vi "LOGIN_rev-1 - Copy.vi"(8 "error in (no error)":errorcluster) -> (0 "error out":errorcluster)   [LabVIEW 2021]
uses:
  Control/login_type.ctl
  Control/User_login_type.ctl
  Control/add_remove.ctl
panel:
  out "Boolean 4":bool=TRUE
  out "element 2":string
  in  "Ring - Menu 8":T1
  in  "Back Button":bool
  out "Boolean 3":bool=TRUE
  out "error in (no error) 4":errorcluster
  in  "error in (no error) 3":errorcluster
  out "Numeric":i32
  out "Enum":T2
  in  "Ring - Menu 7":T1 items=["Admin", "Operator"]
  out "element 3":string
  out "Array 2":string[](array[string])
  in  "Password 3":string
  in  "Enum":T2
  in  "error in (no error) 2":errorcluster
  in  "Remove user":bool
  out "Result":bool
  out "element":string
  out "Ring - Menu 2":u16(ring)
  out "array w/ subset deleted":string[](array[string])
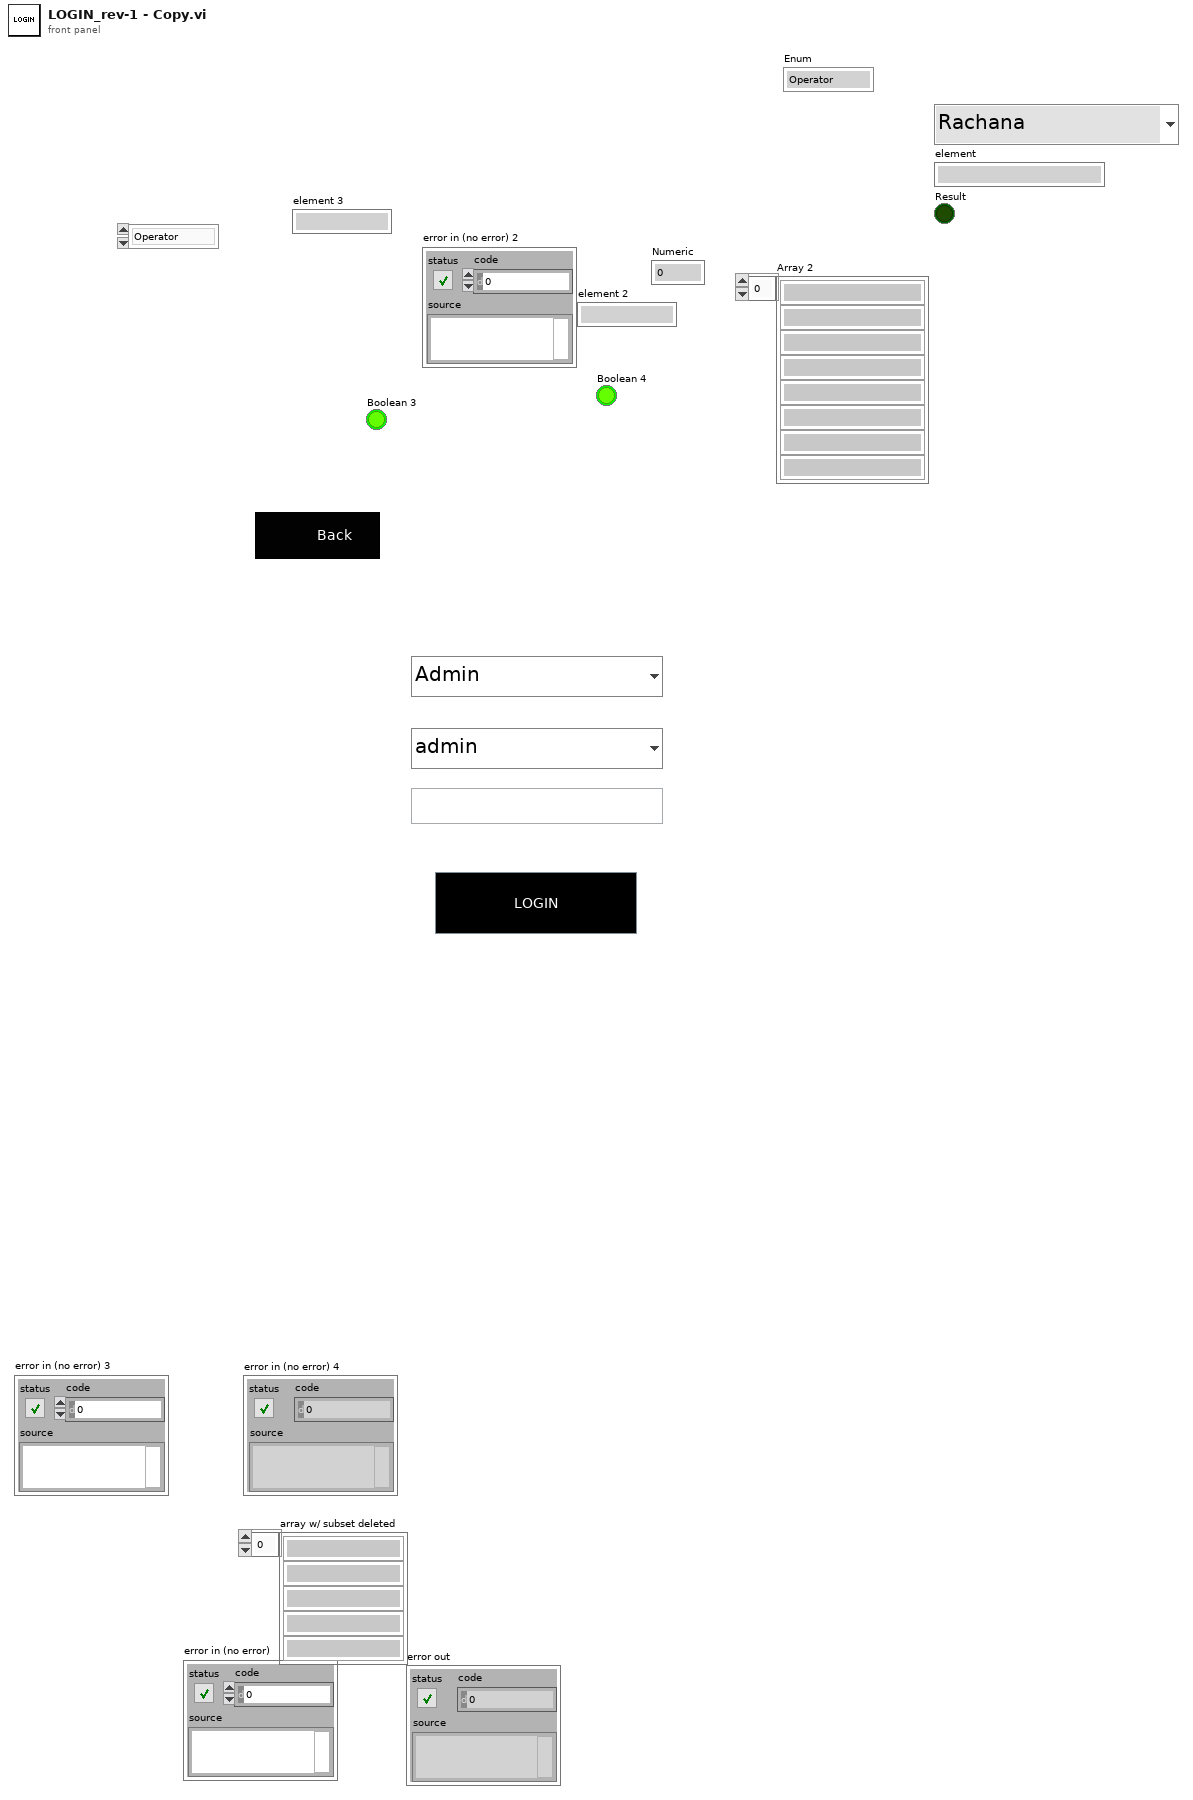
[diagram p1: front panel]
types:
  T1 = typedef "User_login_type.ctl" = u16
  T2 = typedef "login_type.ctl" = enum16{"Operator", "Admin"}
  T3 = typedef "add_remove.ctl" = enum16{"Enter", "add user", "remover user", "view user"}
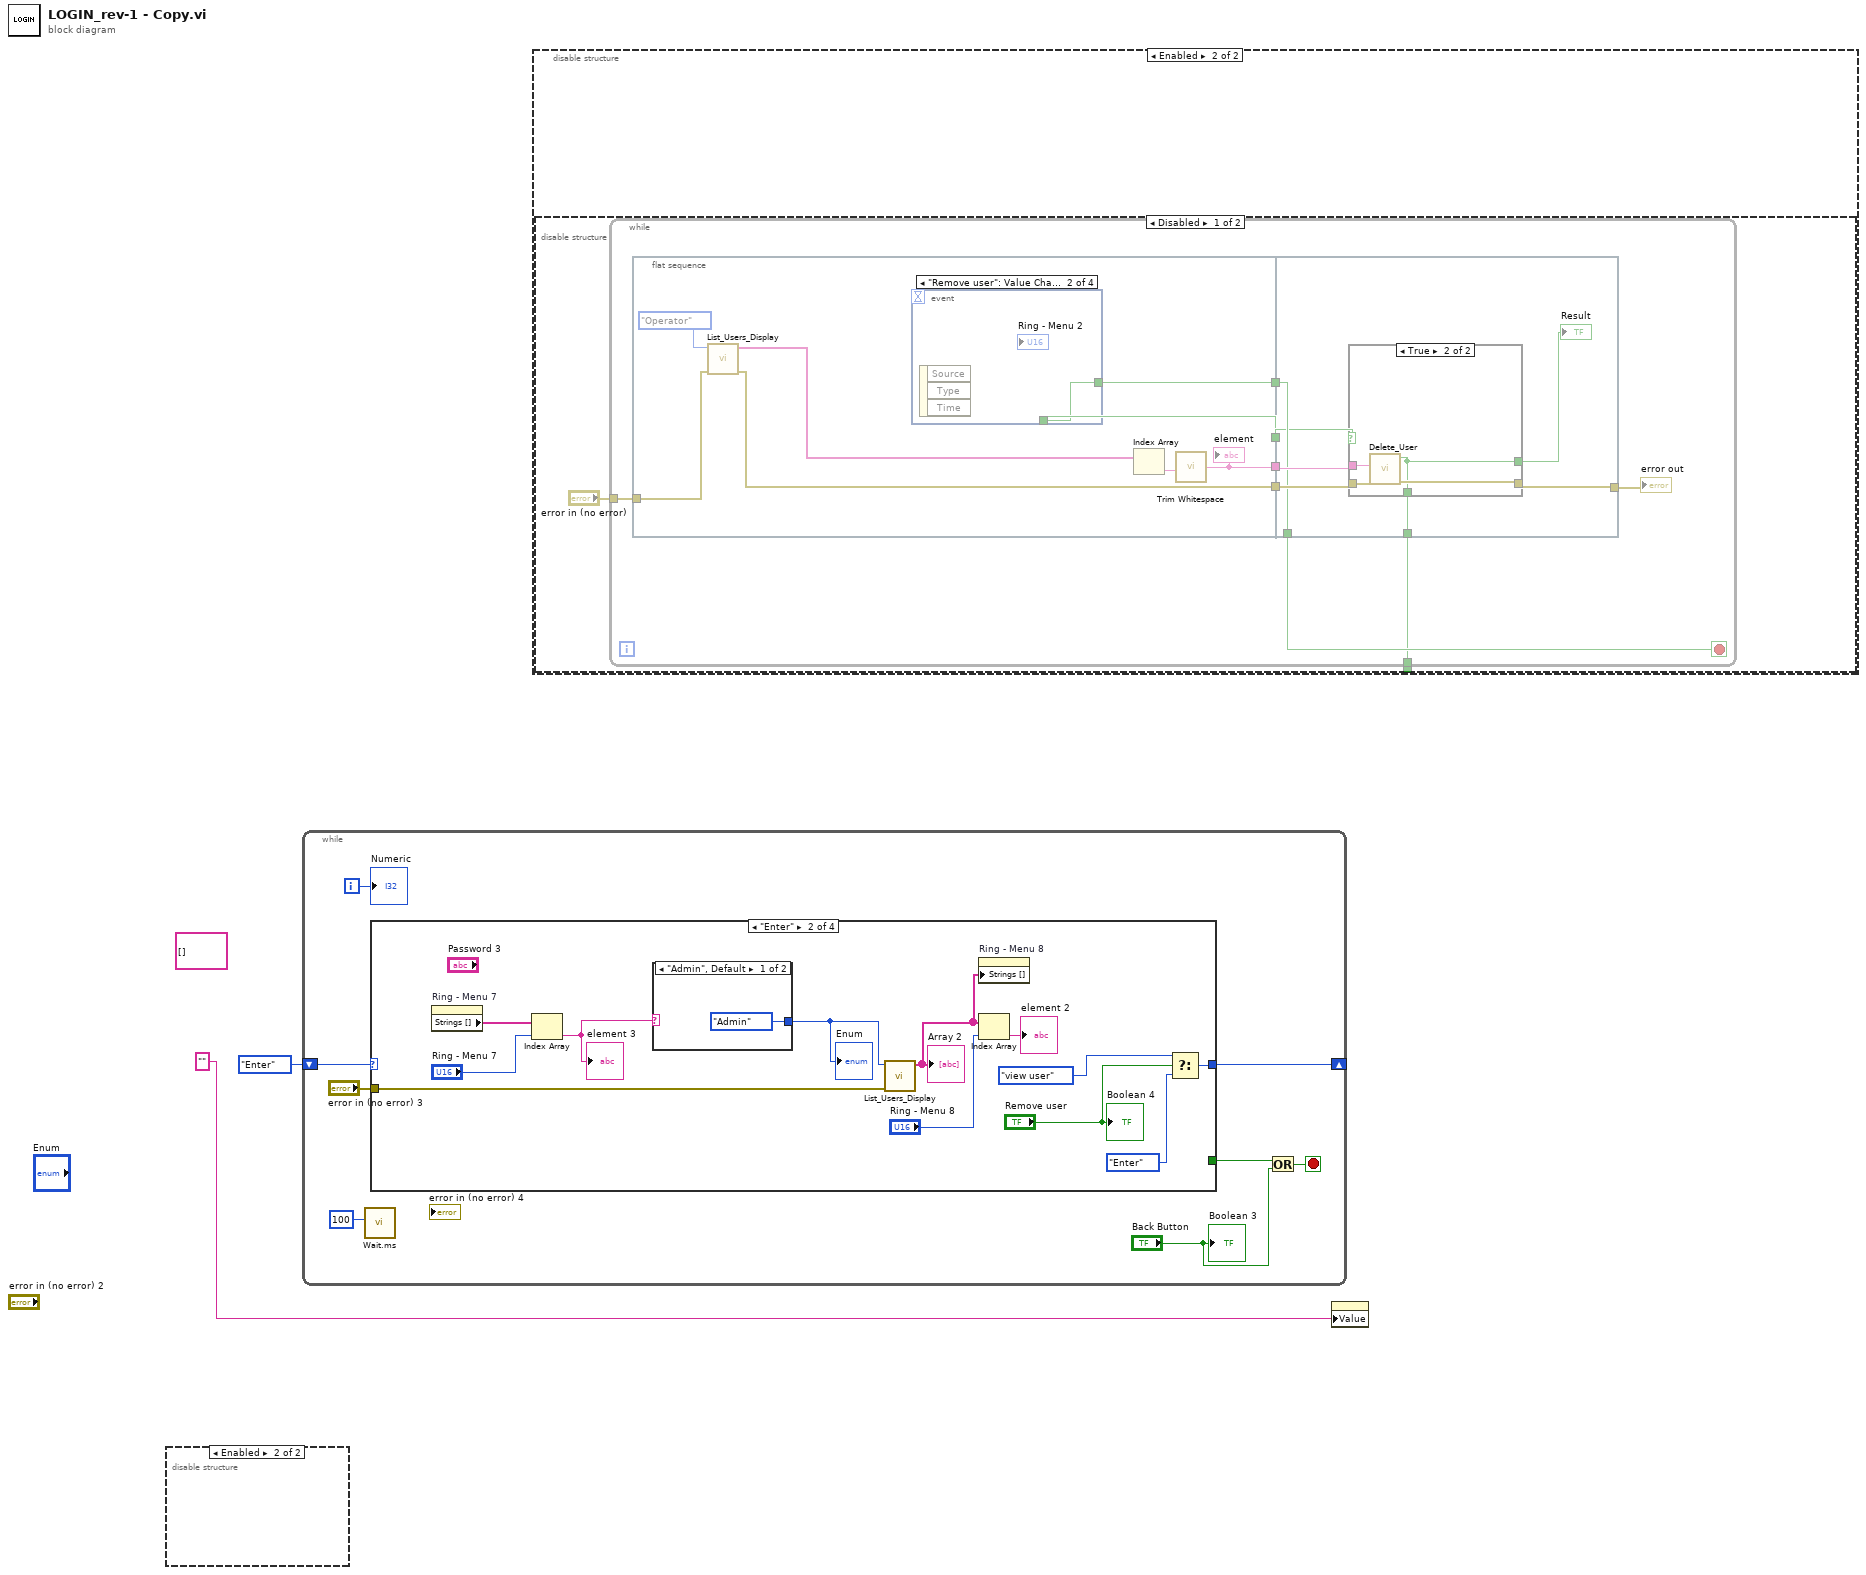
[diagram p0: block diagram]
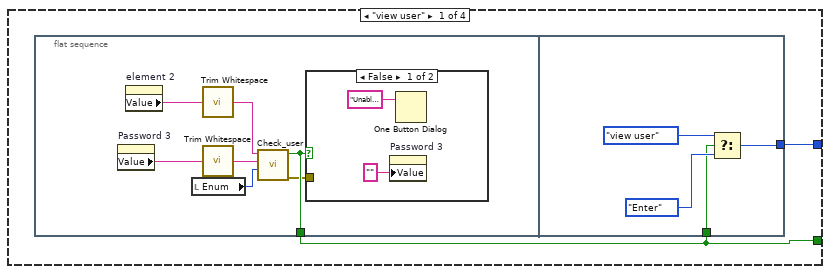
[diagram p2: hidden frame]
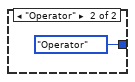
[diagram p4: hidden frame]
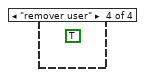
[diagram p6: hidden frame]
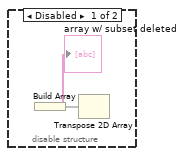
[diagram p8: hidden frame]
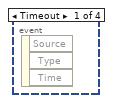
[diagram p9: hidden frame]
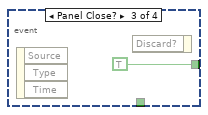
[diagram p10: hidden frame]
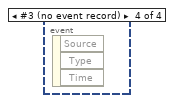
[diagram p11: hidden frame]
diagram:
  (unwired) string[][] [] ("Item Names")
  n1 = disable-structure shown="Enabled" {
    frame Disabled {
    }
    frame Enabled {
    }
  }
  n2 = while {
    shift-right: [w9] -> _
    shift-left: add_remove."Enter" -> [w10]
    i -> [w8]
    stop <- w3 stop-if-true
    n3 = call "Wait.ms.vi"("milliseconds to wait"=u32 100) -> ()  [unwired: 10 in, 1 out]
    n4 = case shown="\"Enter\"" w10 {
      tunnel: [w11 w27 _ _] -> w9
      tunnel: "error in (no error) 3" -> [_ w33 _ _]
      tunnel: [w12 _ _ _] -> w5
      frame "view user" {
        n5 = flat-sequence {
          tunnel: [w18] -> w12
          tunnel: w12 -> [w24]
          tunnel: [w22] -> w11
          frame #0 {
            n6 = property on="Password 3" class="Str"() -> ("Value"=w13:string)  [unwired: 2 in, 2 out]
            n7 = property on="element 2" class="Str"() -> ("Value"=w16:string)  [unwired: 2 in, 2 out]
            n8 = local read "Enum"() -> (w19:T2)
            n9 = call <vilib>:"Trim Whitespace.vi"("string"=w16) -> ("trimmed string"=w15:string)  [unwired: 1 in]
            n10 = call <vilib>:"Trim Whitespace.vi"("string"=w13) -> ("trimmed string"=w14:string)  [unwired: 1 in]
            n11 = call "Check_user.vi"("Enum"=w19, "Password"=w14, "Name"=w15) -> ("error out"=w17:errorcluster, "Result"=w18:bool)  [unwired: 7 in]
            n12 = case shown="False" w18 {
              tunnel: w17 -> [_ _]
              frame False {
                n13 = property on="Password 3" class="Str"("Value"="" ("Password 3")) -> ()  [unwired: 2 in, 2 out]
                n14 = One Button Dialog(message="Unable to login Check ID and password") -> ()  [unwired: 1 in, 1 out]
              }
              frame True {
              }
            }
          }
          frame #1 {
            n15 = Select(t=add_remove."view user", s=w24, f=add_remove."Enter") -> (s? t:f=w22:T3)
          }
        }
      }
      frame "Enter" {
        n16 = property on="Ring - Menu 7" class="Ring (strict)"() -> ("Strings []"=w37:string[])  [unwired: 2 in, 2 out]
        n17 = Index Array(array=w37, index="Ring - Menu 7") -> (element=w35:string)
        "element 3" <- w35
        n18 = case shown="\"Admin\", Default" w35 {
          tunnel: [login_type."Admin" login_type."Operator"] -> w34
          frame "Admin", Default {
          }
          frame "Operator" {
          }
        }
        "Enum" <- w34
        n19 = call "List_Users_Display.vi"("error in (no error)"=w33, "Enum"=w34) -> ("Array"=w32:string[])  [unwired: 8 in, 1 out]
        "Array 2" <- w32
        n20 = property on="Ring - Menu 8" class="Ring (strict)"("Strings []"=w32) -> ()  [unwired: 2 in, 2 out]
        n21 = Index Array(array=w32, index="Ring - Menu 8") -> (element=→"element 2":string)
        n22 = Select(t=add_remove."view user", s="Remove user", f=add_remove."Enter") -> (s? t:f=w27:T3)
        "Boolean 4" <- "Remove user"
      }
      frame "add user" {
      }
      frame "remover user" {
        (unwired) TRUE
      }
    }
    n23 = Or(x=w5, y="Back Button") -> (x .or. y?=w3:bool)
    "Numeric" <- w8
    "Boolean 3" <- "Back Button"
  }
  n24 = disable-structure shown="Enabled" {
    frame Disabled {
      n25 = Build Array("array w/ subset deleted") -> (w40:void[])
      n26 = Transpose 2D Array(2D array=w40) -> (transposed array=w41:void[][])
    }
    frame Enabled {
      n27 = disable-structure shown="Disabled" {
        disable-tunnel: [w43 _] -> _
        frame Disabled {
          n28 = while {
            tunnel: "error in (no error)" -> [w50]
            tunnel: [w45] -> w43
            stop <- w47 stop-if-true
            n29 = flat-sequence {
              tunnel: [w59] -> w52
              tunnel: w50 -> [w56]
              tunnel: [w55] -> w51
              tunnel: [w58] -> w48
              tunnel: [w57] -> w46
              tunnel: w52 -> [w69]
              tunnel: w51 -> [w68]
              tunnel: [w67] -> w49
              tunnel: w48 -> [w66]
              tunnel: [w66] -> w47
              tunnel: w46 -> [w65]
              tunnel: [w63] -> w45
              frame #0 {
                n30 = call "List_Users_Display.vi"("error in (no error)"=w56, "Enum"=login_type."Operator") -> ("error out"=w55:errorcluster, "Array"=w53:string[])  [unwired: 8 in]
                n31 = event shown="[1] \"Remove user\": Value Change" {
                  selector: _ -> [_ _ _ _]
                  dyn-events: _ -> [_ _ _ _]
                  timeout: _ -> [_ _ _ _]
                  tunnel: [_ w61 TRUE _] -> w58
                  tunnel: [_ w61 _ _] -> w57
                  event Timeout {
                    n32 = event-data() -> ()  [unwired: 1 in, 3 out]
                  }
                  event "Remove user": Value Change {
                    n33 = event-data() -> ()  [unwired: 1 in, 3 out]
                  }
                  event Panel Close? {
                    n34 = event-data() -> ()  [unwired: 1 in, 3 out]
                    n35 = event-data() -> ()  [unwired: 2 in, 1 out]
                  }
                  event #3 (no event record) {
                    n36 = event-data() -> ()  [unwired: 1 in, 3 out]
                  }
                }
                n37 = Index Array(array=w53) -> (element=w60:string)  [unwired: 1 in]
                n38 = call <vilib>:"Trim Whitespace.vi"("string"=w60) -> ("trimmed string"=w59:string)  [unwired: 1 in]
                "element" <- w59
              }
              frame #1 {
                n39 = case shown="True" w65 {
                  tunnel: w69 -> [_ w74]
                  tunnel: [_ w71] -> w64
                  tunnel: w68 -> [w70 w73]
                  tunnel: [w70 w72] -> w67
                  tunnel: [_ w71] -> w63
                  frame False {
                  }
                  frame True {
                    n40 = call "Delete_User.vi"("error in (no error)"=w73, "Name"=w74) -> ("error out"=w72:errorcluster, "Result"=w71:bool)  [unwired: 8 in]
                  }
                }
                "Result" <- w64
              }
            }
            "error out" <- w49
          }
        }
        frame Enabled {
        }
      }
    }
  }
  n41 = property on="Password 3" class="Str"("Value"="" ("Name 3")) -> ()  [unwired: 2 in, 2 out]
